vi "Duree rampe temps EPC.vi"(4 "Registre Address":u64, 6 "Unité rampe":u16, 7 "Unit Address (1)":u8, 8 "entrée d'erreur (pas d'erreur)":errorcluster, 9 "Durée":dbl, 11 "Refnum VISA en entrée":refnum<visa-resource-name>) -> (0 "sortie d'erreur":errorcluster, 3 "Refnum VISA en sortie":refnum<visa-resource-name>)   [LabVIEW 2022 SP3]
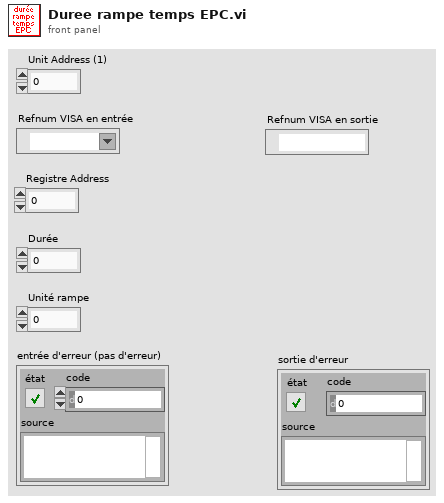
[diagram p1: front panel]
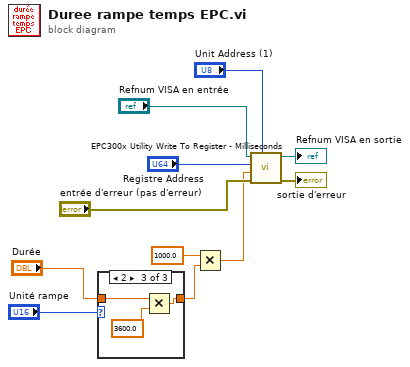
[diagram p0: block diagram]
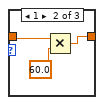
[diagram p3: hidden frame]
diagram:
  n1 = case shown="2" "Unité rampe" {
    tunnel: "Durée" -> [w12 w14 w17]
    tunnel: [w12 w15 w18] -> w2
    frame 0, Default {
    }
    frame 1 {
      n2 = Multiply(x=w14, y=60.0) -> (x*y=w15:dbl)
    }
    frame 2 {
      n3 = Multiply(x=w17, y=3600.0) -> (x*y=w18:dbl)
    }
  }
  n4 = Multiply(x=1000.0, y=w2) -> (x*y=w1:dbl)
  n5 = call "EPC300x Utility Write To Register - Milliseconds.vi"("Unit Address (1)"="Unit Address (1)", "error in (no error)"="entrée d'erreur (pas d'erreur)", "Data in ms (0)"=w1, "Register Address (0)"="Registre Address", "VISA session"="Refnum VISA en entrée") -> ("error out"=→"sortie d'erreur":errorcluster, "dup VISA session"=→"Refnum VISA en sortie":refnum<visa-resource-name>)  [unwired: 5 in]
